vi "ZM-CP-UDP-openReceiver.vi"(8 "error in (no error)":errorcluster, 11 "ZM-CP-communication_protocol in":refnum<class "ZM-CP-communication_protocol.lvclass">) -> (0 "error out":errorcluster, 3 "ZM-CP-communication_protocol out":refnum<class "ZM-CP-communication_protocol.lvclass">)   [LabVIEW 2020, in "ZM-CP-UDP-udp_transport.lvlib" / "ZM-CP-UDP-receiver.lvclass"]
doc: "Hook of the UDP receiver, called by its ZM-CP-init override after Call Parent: opens UDP on localPort (default 61557) and stores the connection. The class terminals are typed as the parent; Preserve Run-Time Class keeps the receiver's class for the override's dynamic output."
uses:
  ZM-CP-UDP-receiver.lvclass
  ZM-CP-communication_protocol/ZM-CP-communication_protocol/ZM-CP-communication_protocol.lvclass
  ZM-CP-UDP-receiver.lvclass/ZM-CP-UDP-receiver.ctl
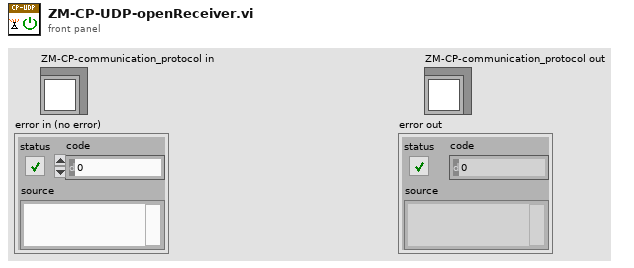
[diagram p1: front panel]
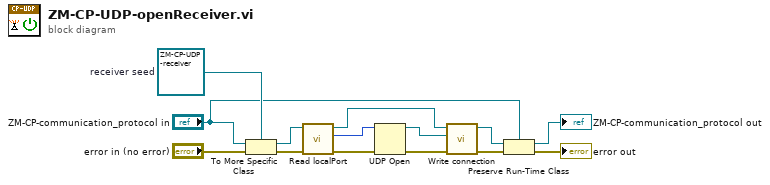
[diagram p0: block diagram]
diagram:
  w13 = refnum<class "ZM-CP-UDP-receiver.lvclass"> refnum  # receiver seed
  n1 = To More Specific Class(target class=w13, reference="ZM-CP-communication_protocol in", error in="error in (no error)") -> (specific class reference=w11:refnum<class "ZM-CP-UDP-receiver.lvclass">, error out=w12:errorcluster)
  n2 = call "Read localPort.vi"("error in (no error)"=w12, "ZM-CP-UDP-receiver in"=w11) -> ("error out"=w9:errorcluster, "localPort"=w10:u16, "ZM-CP-UDP-receiver out"=w7:refnum<class "ZM-CP-UDP-receiver.lvclass">)  [unwired: 7 in]
  n3 = UDP Open(8:w9, 11:w10) -> (port=w6:refnum<k16>, 0:w8:errorcluster)  [unwired: 3 in, 1 out]
  n4 = call "Write connection.vi"("error in (no error)"=w8, "connection"=w6, "ZM-CP-UDP-receiver in"=w7) -> ("error out"=w4:errorcluster, "ZM-CP-UDP-receiver out"=w5:refnum<class "ZM-CP-UDP-receiver.lvclass">)  [unwired: 7 in]
  n5 = Preserve Run-Time Class(object in=w5, error in=w4, 2:"ZM-CP-communication_protocol in") -> (object out=→"ZM-CP-communication_protocol out":refnum<class "ZM-CP-communication_protocol.lvclass">, error out=→"error out":errorcluster)
